vi "License.vi"   [LabVIEW 2014]
doc: "::: VI Helpeks :::\nCopyright (c) 2000-2026 Konstantin Shifershteyn. All rights reserved."
panel:
  # "VI Helpeks\n[EULA]"
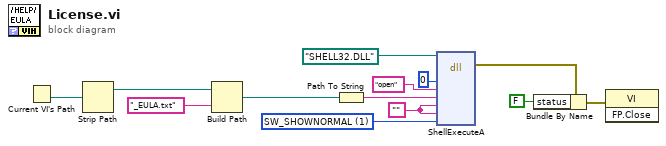
[diagram p0: block diagram]
diagram:
  w5 = 1 items=["SW_HIDE", "SW_SHOWNORMAL", "SW_SHOWMINIMIZED", "SW_SHOWMAXIMIZED", "SW_SHOWNOACTIVE", "SW_SHOW", "SW_MINIMIZE", "SW_SHOWMINNOACTIVE", "SW_SHOWNA", "SW_RESTORE", "SW_SHOWDEFAULT", "SW_FORCEMINIMIZE"] ("show (normal)")
  w10 = ""
  n1 = Current VI's Path() -> (path=w13:path)
  n2 = Strip Path(path=w13) -> (stripped path=w12:path)  [unwired: 1 out]
  n3 = Build Path(base path=w12, name or relative path="_EULA.txt") -> (appended path=w6:path)
  n4 = Path To String(path=w6) -> (string=w8:string)
  n5 = dll-call lib="SHELL32.DLL" fn="ShellExecuteA"(path in=path "SHELL32.DLL", "hWnd"=0, "Operation"="open", "File"=w8, "Parameters"=w10, "DefaultDir"=w10, "ShowCmd"=w5) -> (error out=w4:errorcluster)  [unwired: 9 in, 1 out]
  n6 = Bundle By Name(cluster=w4, "status"=FALSE) -> (w3:errorcluster)
  n7 = invoke class="VI" method="FP.Close"(error in=w3) -> ()  [unwired: 2 in, 3 out]
